vi "Device_Status.vi"(8 "error in (no error)":errorcluster, 11 "CANsub_DirectChannel in":refnum<class "CANsub_DirectChannel.lvclass">) -> (0 "error out":errorcluster, 2 "device status":T1, 3 "CANsub_DirectChannel out":refnum<class "CANsub_DirectChannel.lvclass">)   [LabVIEW 2021, in "CANsub_API.lvlib" / "CANsub_DirectChannel.lvclass"]
doc: "Reads the CAN controller state and the error counters from the device with one REST call. The HTTPS client stays open between calls: the first call takes about 80 ms, a later call about 1 ms. It does not use the WebSocket connection."
uses:
  CANsub_DirectChannel.lvclass
  CANsub_DirectChannel.lvclass/CANsub_DirectChannel.ctl
  CANsub_API.lvlib
  common/Typedefs/CANsub_Device_Status.ctl
  common/CANsub_Common.lvlib
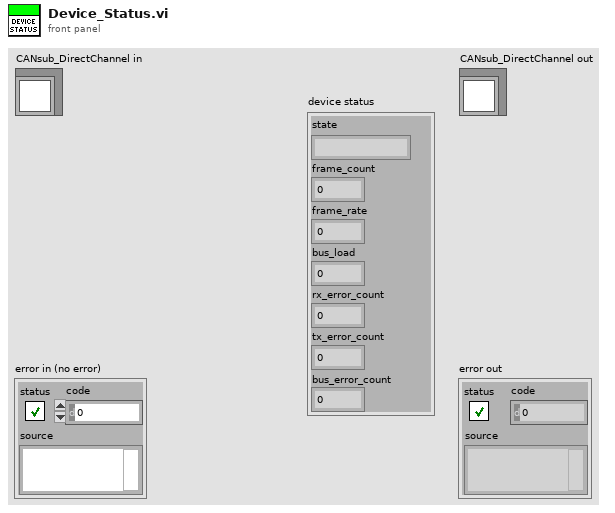
[diagram p1: front panel]
types:
  T1 = typedef "CANsub_Common.lvlib/CANsub_Device_Status.ctl" = cluster{"state":string, "frame_count":u32, "frame_rate":dbl, "bus_load":dbl, "rx_error_count":u32, "tx_error_count":u32, "bus_error_count":u32}
  T2 = typedef "CANsub_Common.lvlib/CANsub_connection.ctl" = cluster{"host":string, "channel":u8, "cert path":path}
  T3 = typedef "LabVIEWHTTPClient.lvlib/ClientHandle.ctl" = refnum<k1>
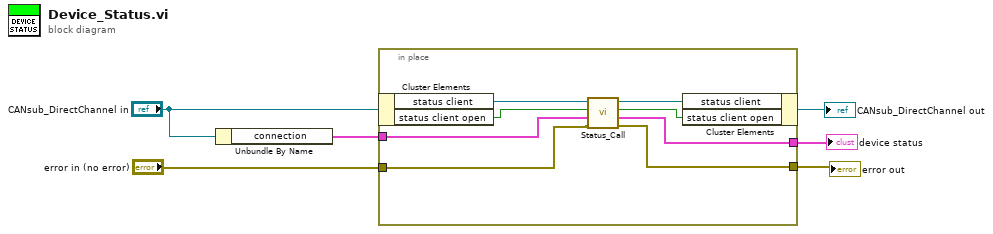
[diagram p0: block diagram]
diagram:
  n1 = Unbundle By Name("CANsub_DirectChannel in") -> ("connection"=w5:T2)
  n2 = in-place {
    in-place-border: w5 -> [w14]
    in-place-border: "error in (no error)" -> [w11]
    in-place-border: [w8] -> w2
    in-place-border: [w7] -> w3
    n3 = in-place-cluster #1("CANsub_DirectChannel in") -> ("status client"=w13:T3, "status client open"=w12:bool)
    n4 = call "Status_Call.vi"("error in (no error)"=w11, "connection"=w14, "open in"=w12, "status client in"=w13) -> ("error out"=w8:errorcluster, "device status"=w7:T1, "open out"=w9:bool, "status client out"=w10:T3)  [unwired: 4 in]
    n5 = in-place-cluster #1("status client"=w10, "status client open"=w9) -> (→"CANsub_DirectChannel out":refnum<class "CANsub_DirectChannel.lvclass">)
  }
  "error out" <- w2
  "device status" <- w3
